vi "Enqueue_Message.vi"(7 "Priority Message? (F)":bool, 8 "error in (no error)":errorcluster={"status"=FALSE, "code"=0, "source"="\"\""}, 9 "Message Data":string, 10 "Message":string) -> (0 "error out":errorcluster, 3 "Message Cluster":cluster{"Message":string, "Message Data":string})   [LabVIEW 2026]
doc: "For a regular message, enqueue the message. For a priority message, enqueue it at the front of the queue."
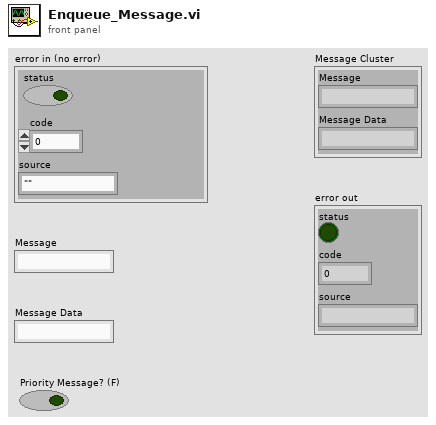
[diagram p1: front panel]
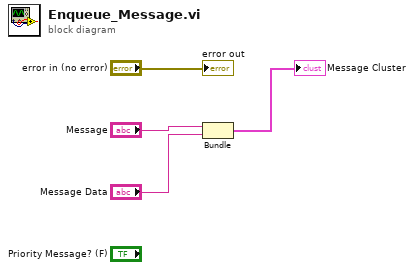
[diagram p0: block diagram]
diagram:
  n1 = Bundle("Message"="Message", "Message Data"="Message Data") -> (→"Message Cluster":cluster{"Message":string, "Message Data":string})  [unwired: 1 in]
  "error out" <- "error in (no error)"
